vi "Close FP if in LabVIEW Dir.vi"(7 "VI Refnum":refnum<vi>, 8 "Error in":errorcluster caption="Error in (no error)") -> (0 "Error out":errorcluster)   [LabVIEW 2017, in "csm-ui-support.lvlib"]
uses:
  csm-ui-support.lvlib
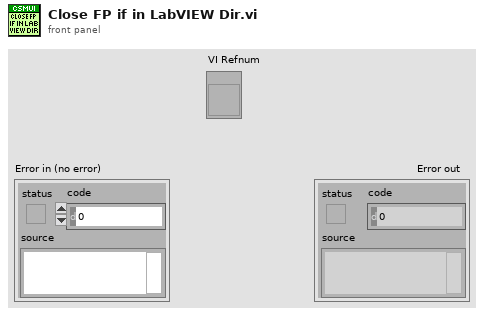
[diagram p1: front panel]
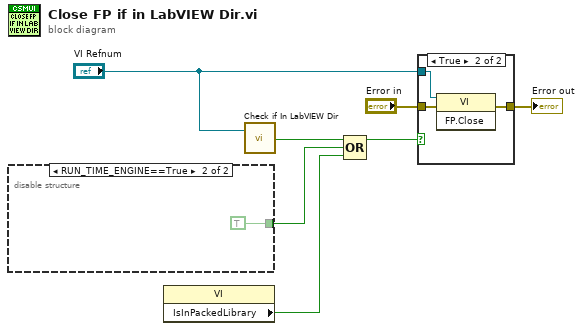
[diagram p0: block diagram]
diagram:
  n1 = disable-structure shown="RUN_TIME_ENGINE==True" {
    disable-tunnel: [_ TRUE] -> w2
    frame condition #0 (active) {
    }
    frame condition #1 {
    }
  }
  n2 = property class="VI"() -> ("IsInPackedLibrary"=w1:bool)  [unwired: 2 in, 2 out]
  n3 = call "Check if In LabVIEW Dir.vi"("VI Refnum"="VI Refnum") -> ("Boolean"=w7:bool)  [unwired: 1 in]
  n4 = Compound Arithmetic op=OR(w7, w2, w1) -> (w3:bool)
  n5 = case shown="True" w3 {
    tunnel: [w9 w12] -> w6
    tunnel: "Error in" -> [w9 w11]
    tunnel: "VI Refnum" -> [_ w10]
    frame False {
    }
    frame True {
      n6 = invoke class="VI" method="FP.Close"(reference=w10, error in=w11) -> (error out=w12:errorcluster)  [unwired: 1 in, 2 out]
    }
  }
  "Error out" <- w6
